vi "Start CSM DebugTool Dialog.vi"(8 "error in (no error)":errorcluster, 11 "Application In":refnum<vi>) -> (0 "error out":errorcluster)   [LabVIEW 2017, in "CSM DebugTool Dialog.lvlib"]
uses:
  CSM DebugTool Dialog.lvlib
  _Shared/CSM Shared.lvlib
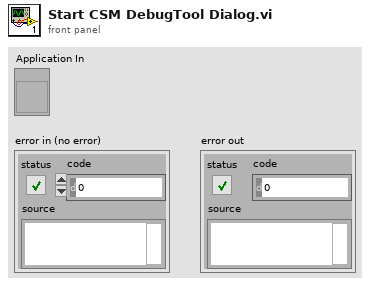
[diagram p1: front panel]
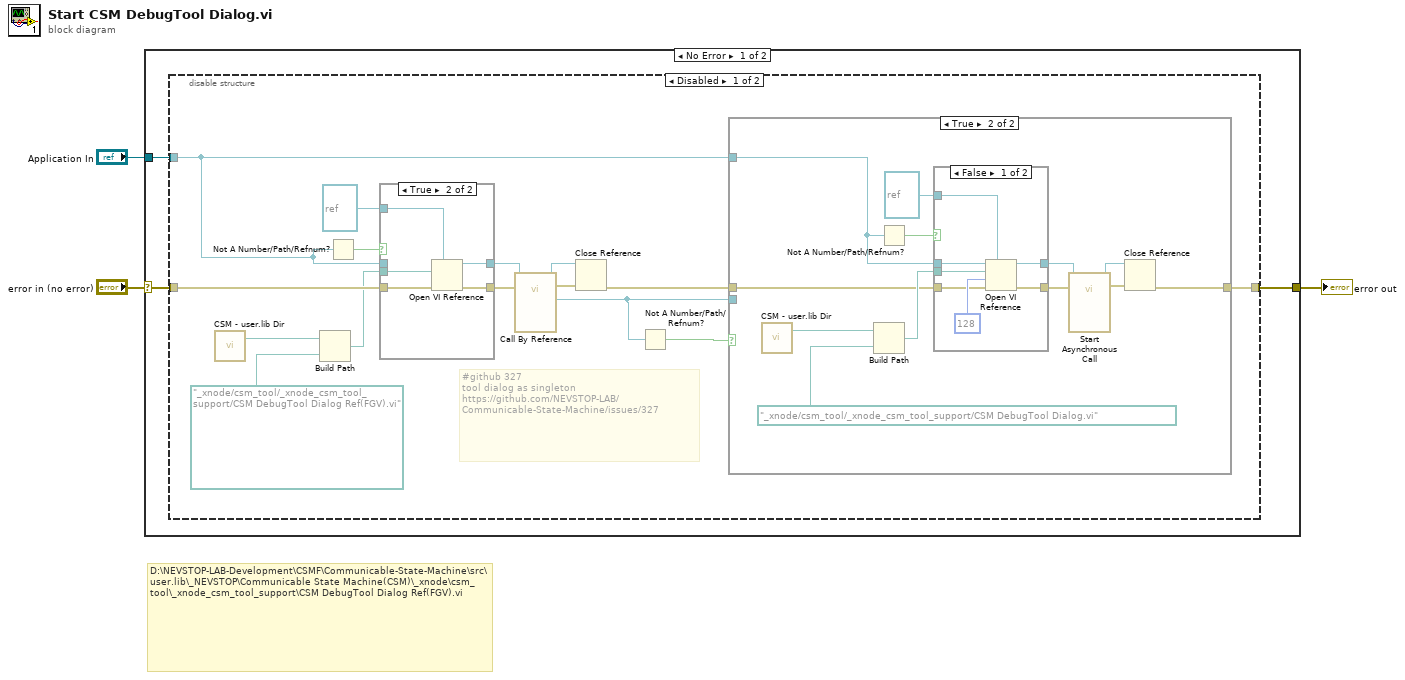
[diagram p0: block diagram]
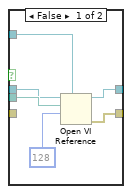
[diagram p2: hidden frame]
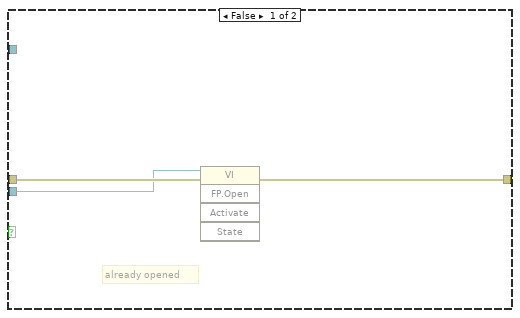
[diagram p3: hidden frame]
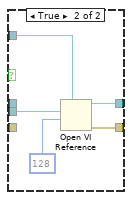
[diagram p4: hidden frame]
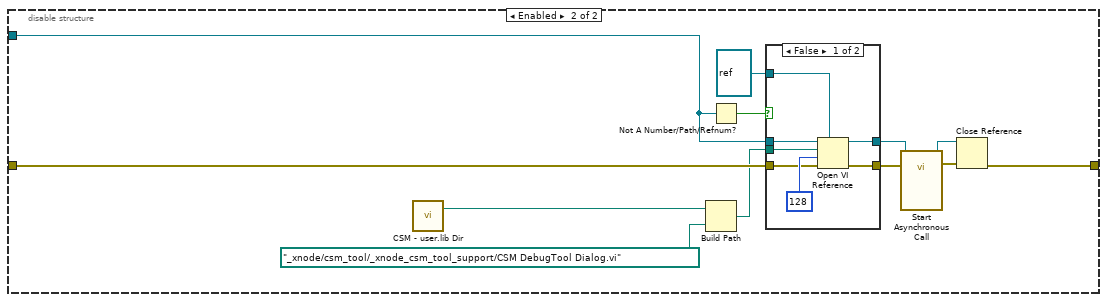
[diagram p5: hidden frame]
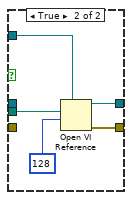
[diagram p6: hidden frame]
diagram:
  # "D:\\NEVSTOP-LAB-Development\\CSMF\\Communicable-State-Machine\\src\\user.lib\\_NEVSTOP\\Communicable State Machine(CSM)\\_xnode\\csm_tool\\_xnode_csm_tool_support\\CSM DebugTool Dialog Ref(FGV).vi"
  n1 = case shown="No Error" "error in (no error)" {
    selector: "error in (no error)" -> [w5 w84]
    tunnel: [w6 w84] -> w3
    tunnel: "Application In" -> [w4 _]
    frame No Error {
      n2 = disable-structure shown="Disabled" {
        disable-tunnel: [w21 w71] -> w6
        disable-tunnel: w5 -> [w20 w70]
        disable-tunnel: w4 -> [w18 w69]
        frame Disabled {
          # "#github 327 \ntool dialog as singleton\nhttps://github.com/NEVSTOP-LAB/Communicable-State-Machine/issues/327"
          n3 = call "CSM - user.lib Dir.vi"() -> ("csm_user.lib_dir"=w10:path)  [unwired: 2 in, 1 out]
          n4 = Build Path(base path=w10, name or relative path=path "_xnode/csm_tool/_xnode_csm_tool_support/CSM DebugTool Dialog Ref(FGV).vi") -> (appended path=w11:path)
          n5 = Not A Number/Path/Refnum?(number/path/refnum=w18) -> (NaN/Path/Refnum?=w9:bool)
          n6 = case shown="True" w9 {
            tunnel: [w27 w32] -> w13
            tunnel: [w26 w31] -> w12
            tunnel: w11 -> [w25 w30]
            tunnel: w18 -> [w23 _]
            tunnel: refnum<vi> refnum ("type specifier VI Refnum (for type only)") -> [w22 w29]
            tunnel: w20 -> [_ w28]
            frame False {
              n7 = Open VI Reference(type specifier VI Refnum (for type only)=w22, application reference (local)=w23, vi path=w25, options=128) -> (vi reference=w27:refnum<vi>, error out=w26:errorcluster)  [unwired: 2 in]
            }
            frame True {
              n8 = Open VI Reference(type specifier VI Refnum (for type only)=w29, vi path=w30, error in (no error)=w28) -> (vi reference=w32:refnum<vi>, error out=w31:errorcluster)  [unwired: 3 in]
            }
          }
          n9 = call-by-ref "?"(reference=w13, error in=w12) -> (reference out=w15:refnum<vi>, error out=w14:errorcluster, "VI Reference(out)"=w16:refnum<vi>)  [unwired: 11 in]
          n10 = Close Reference(reference=w15, error in (no error)=w14) -> (error out=w17:errorcluster)
          n11 = Not A Number/Path/Refnum?(number/path/refnum=w16) -> (NaN/Path/Refnum?=w19:bool)
          n12 = case shown="True" w19 {
            tunnel: [w35 w41] -> w21
            tunnel: w18 -> [_ w39]
            tunnel: w17 -> [w34 w37]
            tunnel: w16 -> [w33 _]
            frame False {
              # "already opened"
              n13 = invoke class="VI" method="FP.Open"(reference=w33, error in=w34) -> (error out=w35:errorcluster)  [unwired: 3 in, 4 out]
            }
            frame True {
              n14 = call "CSM - user.lib Dir.vi"() -> ("csm_user.lib_dir"=w42:path)  [unwired: 2 in, 1 out]
              n15 = Build Path(base path=w42, name or relative path=path "_xnode/csm_tool/_xnode_csm_tool_support/CSM DebugTool Dialog.vi") -> (appended path=w43:path)
              n16 = Not A Number/Path/Refnum?(number/path/refnum=w39) -> (NaN/Path/Refnum?=w40:bool)
              n17 = case shown="False" w40 {
                tunnel: [w54 w59] -> w45
                tunnel: [w53 w58] -> w44
                tunnel: w43 -> [w52 w57]
                tunnel: w39 -> [w50 _]
                tunnel: refnum<vi> refnum ("type specifier VI Refnum (for type only)") -> [w49 w55]
                tunnel: w37 -> [w48 _]
                frame False {
                  n18 = Open VI Reference(type specifier VI Refnum (for type only)=w49, application reference (local)=w50, vi path=w52, options=128, error in (no error)=w48) -> (vi reference=w54:refnum<vi>, error out=w53:errorcluster)  [unwired: 1 in]
                }
                frame True {
                  n19 = Open VI Reference(type specifier VI Refnum (for type only)=w55, vi path=w57, options=128) -> (vi reference=w59:refnum<vi>, error out=w58:errorcluster)  [unwired: 3 in]
                }
              }
              n20 = call-by-ref "Start Asynchronous Call"(reference=w45, error in=w44) -> (reference out=w47:refnum<vi>, error out=w46:errorcluster)  [unwired: 12 in]
              n21 = Close Reference(reference=w47, error in (no error)=w46) -> (error out=w41:errorcluster)
            }
          }
        }
        frame Enabled {
          n22 = call "CSM - user.lib Dir.vi"() -> ("csm_user.lib_dir"=w63:path)  [unwired: 2 in, 1 out]
          n23 = Build Path(base path=w63, name or relative path=path "_xnode/csm_tool/_xnode_csm_tool_support/CSM DebugTool Dialog.vi") -> (appended path=w64:path)
          n24 = Not A Number/Path/Refnum?(number/path/refnum=w69) -> (NaN/Path/Refnum?=w62:bool)
          n25 = case shown="False" w62 {
            tunnel: [w78 w83] -> w66
            tunnel: [w77 w82] -> w65
            tunnel: w64 -> [w76 w81]
            tunnel: w69 -> [w74 _]
            tunnel: refnum<vi> refnum ("type specifier VI Refnum (for type only)") -> [w73 w79]
            tunnel: w70 -> [w72 _]
            frame False {
              n26 = Open VI Reference(type specifier VI Refnum (for type only)=w73, application reference (local)=w74, vi path=w76, options=128, error in (no error)=w72) -> (vi reference=w78:refnum<vi>, error out=w77:errorcluster)  [unwired: 1 in]
            }
            frame True {
              n27 = Open VI Reference(type specifier VI Refnum (for type only)=w79, vi path=w81, options=128) -> (vi reference=w83:refnum<vi>, error out=w82:errorcluster)  [unwired: 3 in]
            }
          }
          n28 = call-by-ref "Start Asynchronous Call"(reference=w66, error in=w65) -> (reference out=w68:refnum<vi>, error out=w67:errorcluster)  [unwired: 12 in]
          n29 = Close Reference(reference=w68, error in (no error)=w67) -> (error out=w71:errorcluster)
        }
      }
    }
    frame Error {
    }
  }
  "error out" <- w3
